vi "Add Language to Controls.vi"(7 "ANSI":bool, 11 "Translastions in":map{string, T1}(c390)) -> (3 "Translastions out":map{string, T1}(c390))   [LabVIEW 2019, in "Language Editor.lvlib"]
doc: "- - -\nCopyright (c) 2026, Merecs Engineering GmbH"
uses:
  Language Editor.lvlib
  type defs/Cluster Translations.ctl
  Language Selection/TypeDefs/Cluster PropertyTranslation.ctl
  Language Selection/TypeDefs/Enum Property Type.ctl
  Language Selection/Language Selection.lvlib
panel:
  # "Connector Pane"
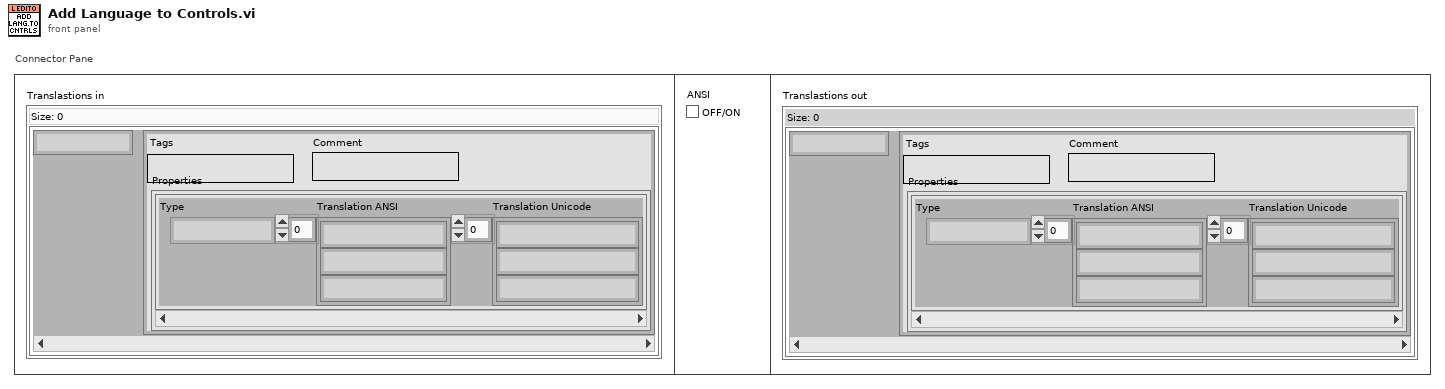
[diagram p1: front panel]
types:
  T1 = typedef "Language Editor.lvlib/Cluster Translations.ctl" = cluster{"Tags":string, "Comment":string, "Properties":T2[]}
  T2 = typedef "Language Selection.lvlib/Cluster PropertyTranslation.ctl" = cluster{"Type":T3, "Translation ANSI":string[], "Translation Unicode":string[]}
  T3 = typedef "Language Selection.lvlib/Enum Property Type.ctl" = enum16{"NA", "Caption", "String Value", "Boolean Text", "Ring Strings", "1D Array Elements", "2D Array Elements", "(MC)Listbox Header", "(MC)Listbox Items", "Tab Pages Names", "X & Y GraphChart", "Plot Names", "Table Headers", "Table Items", "TipStrip", "Combobox Strings", "Cursor Name", "Tree Col Headers"}
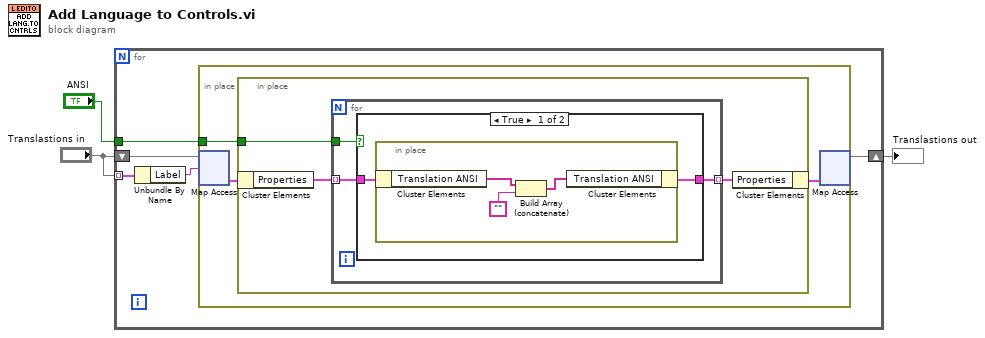
[diagram p0: block diagram]
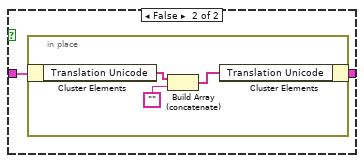
[diagram p2: hidden frame]
diagram:
  n1 = for {
    tunnel: "Translastions in" -> [w7] mode=indexing
    tunnel: "ANSI" -> [w5]
    shift-right: [w4] -> w1
    shift-left: "Translastions in" -> [w8]
    n2 = Unbundle By Name(w7) -> ("Label"=w6:string)
    n3 = in-place {
      in-place-border: w5 -> [w11]
      n4 = in-place-map #1(w8, w6) -> (w10:T1)  [unwired: 1 in, 1 out]
      n5 = in-place {
        in-place-border: w11 -> [w14]
        n6 = in-place-cluster #2(w10) -> ("Properties"=w13:T2[])
        n7 = for {
          tunnel: w13 -> [w16] mode=indexing
          tunnel: [w17] -> w12 mode=indexing
          tunnel: w14 -> [w15]
          n8 = case shown="True" w15 {
            tunnel: [w19 w24] -> w17
            tunnel: w16 -> [w18 w23]
            frame True {
              n9 = in-place {
                n10 = in-place-cluster #3(w18) -> ("Translation ANSI"=w22:string[])
                n11 = Build Array (concatenate)(w22, "") -> (w21:string[])
                n12 = in-place-cluster #3("Translation ANSI"=w21) -> (w19:T2)
              }
            }
            frame False {
              n13 = in-place {
                n14 = in-place-cluster #4(w23) -> ("Translation Unicode"=w27:string[])
                n15 = Build Array (concatenate)(w27, "") -> (w26:string[])
                n16 = in-place-cluster #4("Translation Unicode"=w26) -> (w24:T2)
              }
            }
          }
        }
        n17 = in-place-cluster #2("Properties"=w12) -> (w9:T1)
      }
      n18 = in-place-map #1(w9) -> (w4:map{string, T1})  [unwired: 1 in, 2 out]
    }
  }
  "Translastions out" <- w1
